vi "LTE Configure ModAcc.vi"(0 "RFmx Handle In":refnum<k21>, 1 "Selector String":string, 5 "ModAcc Configuration":T1={"Synchronization Mode"=1, "Measurement Offset"=0, "Measurement Length"=1, "EVM Unit"=0, "Averaging Enabled"=0, "Averaging Count"=10} {"Averaging Enabled" items=["False", "True"]; "EVM Unit" items=["Percentage", "dB"]; "Synchronization Mode" items=["Frame", "Slot", "Marker"]}, 11 "error in (no error)":errorcluster) -> (4 "RFmx Handle Out":refnum<k21>, 15 "error out":errorcluster)   [LabVIEW 2016, in "RFmxLTE.lvlib"]
doc: "Configures common settings for the ModAcc measurement and selects the measurement."
uses:
  RFmxLTE.lvlib
  Typedefs/LTE ModAcc Configuration.ctl
  <vilib>/RFmx/LTE/mx/RFmxLTE.llb/RFmxLTE Select Measurement (Single).vi
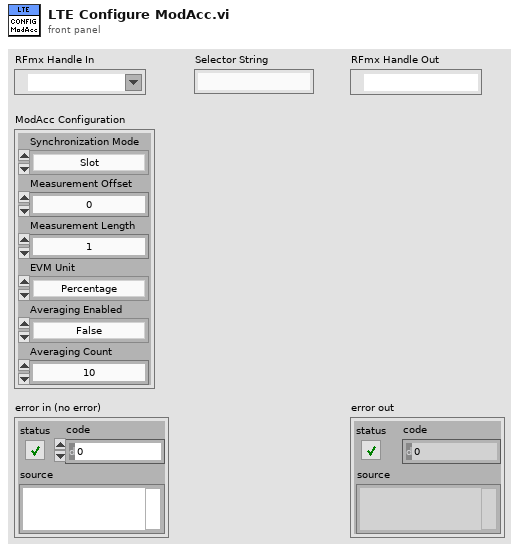
[diagram p1: front panel]
types:
  T1 = typedef "RFmxLTE.lvlib/LTE ModAcc Configuration.ctl" = cluster{"Synchronization Mode":i32, "Measurement Offset":i32, "Measurement Length":i32, "EVM Unit":i32, "Averaging Enabled":i32, "Averaging Count":i32}
  T2 = enum16{"ACP", "CHP", "ModAcc", "OBW", "SEM", "PVT", "SlotPhase", "SlotPower"}
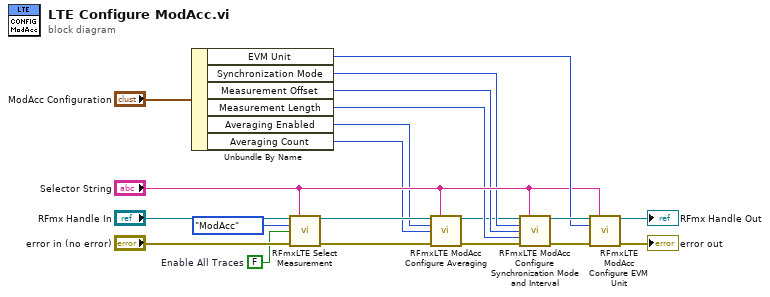
[diagram p0: block diagram]
diagram:
  w7 = FALSE  # Enable All Traces
  n1 = Unbundle By Name("ModAcc Configuration") -> ("EVM Unit"=w13:i32, "Synchronization Mode"=w6:i32, "Measurement Offset"=w5:i32, "Measurement Length"=w4:i32, "Averaging Enabled"=w3:i32, "Averaging Count"=w2:i32)
  n2 = call-poly <vilib>:"RFmxLTE Select Measurement.vi"("Instrument Handle In"="RFmx Handle In", "Selector String"="Selector String", "Measurement"=T2."ModAcc", "Enable All Traces"=w7, "error in (no error)"="error in (no error)") -> ("Instrument Handle Out"=w12:refnum<k21>, "error out"=w17:errorcluster)  [unwired: 9 in]
  n3 = call <vilib>:"RFmxLTE ModAcc Configure Averaging.vi"("Instrument Handle In"=w12, "Selector String"="Selector String", "Averaging Enabled"=w3, "Averaging Count"=w2, "error in (no error)"=w17) -> ("Instrument Handle Out"=w1:refnum<k21>, "error out"=w20:errorcluster)  [unwired: 9 in]
  n4 = call <vilib>:"RFmxLTE ModAcc Configure Synchronization Mode and Interval.vi"("Instrument Handle In"=w1, "Selector String"="Selector String", "Synchronization Mode"=w6, "Measurement Offset (slots)"=w5, "Measurement Length (slots)"=w4, "error in (no error)"=w20) -> ("Instrument Handle Out"=w15:refnum<k21>, "error out"=w19:errorcluster)  [unwired: 8 in]
  n5 = call <vilib>:"RFmxLTE ModAcc Configure EVM Unit.vi"("Instrument Handle In"=w15, "Selector String"="Selector String", "EVM Unit"=w13, "error in (no error)"=w19) -> ("Instrument Handle Out"=→"RFmx Handle Out":refnum<k21>, "error out"=→"error out":errorcluster)  [unwired: 10 in]
